vi "ExecuteCommand.vi"(0 "reference in":refnum<class "DqmhModuleDiagramGraph.lvclass">, 1 "CommandData":variant, 2 "selected":T1, 3 "selectedEdge":refnum<class "AbstractEdge.lvclass">, 4 "SelectedNodes":refnum<class "AbstractNode.lvclass">[](array[class]), 5 "error in (no error)":errorcluster) -> (14 "reference out":refnum<class "DqmhModuleDiagramGraph.lvclass">, 15 "Cancelled":bool, 19 "error out":errorcluster)   [LabVIEW 2020, in "DqmhModuleDiagramGraph.lvclass"]
uses:
  <resource>/Framework/Providers/Open_GDS/UML/DqmhModuleDiagramGraph_class/DqmhModuleDiagramGraph.lvclass
  <resource>/Framework/Providers/Open_GDS/UML/AbstractNode_class/AbstractNode.lvclass
  <resource>/Framework/Providers/Open_GDS/UML/AbstractEdge_class/AbstractEdge.lvclass
  <resource>/Framework/Providers/Open_GDS/UML/UMLEditor/UMLEditor tooltype.ctl
  <resource>/Framework/Providers/Open_GDS/UML/DQMHModuleNode_class/DQMHModuleNode.lvclass
  <resource>/Framework/Providers/Open_GDS/UML/DQMHModuleNode_class/ExternalSetTypes.ctl
  <resource>/Framework/Providers/Open_GDS/UML/DQMH_API_class/DQMH_API.lvclass
panel:
  out "StatusText":string
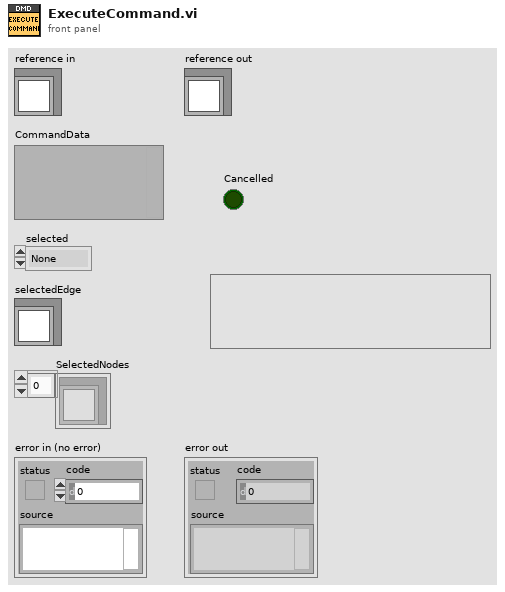
[diagram p1: front panel]
types:
  T1 = typedef "UMLEditor tooltype.ctl" = enum16{"None", "Node", "Edge"}
  T2 = enum32{"Invalid", "Standard", "Closed", "Hidden", "Minimized", "Maximized"}
  T3 = enum32{"Invalid", "Default", "Floating", "Floating/Auto-Hide", "Modal"}
  T4 = typedef "DQMHModuleNode.lvclass/ExternalSetTypes.ctl" = enum16{"Name", "Attributes", "Methods", "Position", "ShowEvents", "ShowInternalData", "ClassPath"}
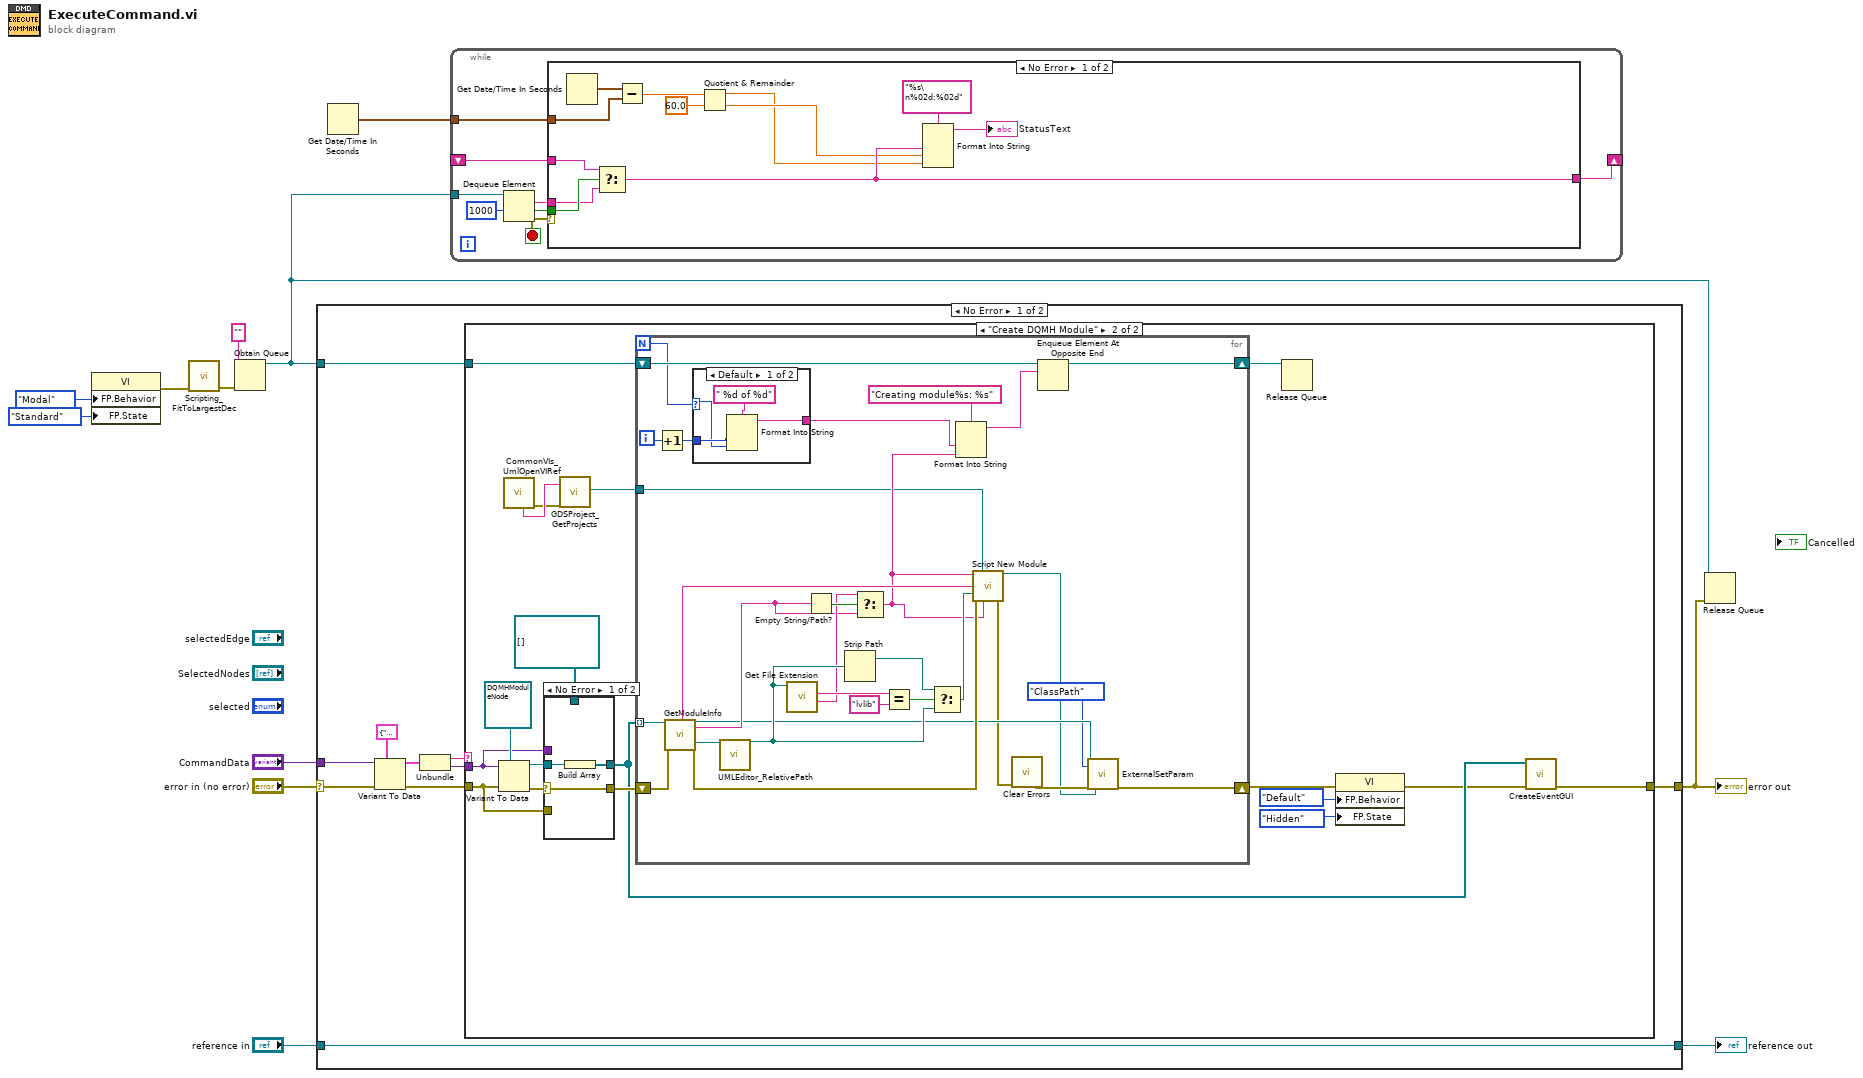
[diagram p0: block diagram]
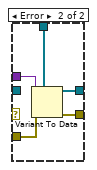
[diagram p4: hidden frame]
diagram:
  n1 = property class="VI"("FP.Behavior"=T3."Modal" ("Front Panel Window:Behavior"), "FP.State"=T2."Standard" ("Front Panel Window:State")) -> (error out=w2:errorcluster)  [unwired: 2 in, 1 out]
  n2 = call <resource>:"Scripting_FitToLargestDec.vi"("error in (no error)"=w2) -> ("error out"=w8:errorcluster)  [unwired: 5 in, 1 out]
  n3 = Obtain Queue(element data type="" ("y"), error in (no error)=w8) -> (queue out=w6:refnum<queue>)  [unwired: 3 in, 2 out]
  n4 = case shown="No Error" "error in (no error)" {
    selector: "error in (no error)" -> [w19 w85]
    tunnel: [w15 w85] -> w7
    tunnel: [w22 w84] -> w10
    tunnel: "reference in" -> [w22 w84]
    tunnel: "CommandData" -> [w20 _]
    tunnel: w6 -> [w13 _]
    frame No Error {
      n5 = Variant To Data(error in=w19, type=cluster{"Cmd":string, "Data":variant} {"Cmd"="", "Data"=variant} ("FlattenCommandSettings"), Variant=w20) -> (data=w18:cluster{"Cmd":string, "Data":variant}, error out=w16:errorcluster)
      n6 = Unbundle(w18) -> ("Cmd"=w17:string, "Data"=w14:variant)
      n7 = case shown="\"Create DQMH Module\"" w17 {
        tunnel: w16 -> [w23 w34]
        tunnel: [w23 w25] -> w15
        tunnel: w14 -> [_ w35]
        tunnel: w13 -> [_ w39]
        frame Default {
        }
        frame "Create DQMH Module" {
          n8 = Variant To Data(error in=w34, type=refnum<class "DQMHModuleNode.lvclass"> refnum ("DQMHModuleNode"), Variant=w35) -> (data=w40:refnum<class "DQMHModuleNode.lvclass">, error out=w38:errorcluster)
          n9 = call <resource>:"CommonVIs_UmlOpenVIRef.vi"() -> ("error out"=w32:errorcluster, "ProjectNameOut"=w33:string)  [unwired: 4 in, 6 out]
          n10 = case shown="No Error" w38 {
            selector: w38 -> [w42 _]
            tunnel: w40 -> [w44 _]
            tunnel: [w43 w45] -> w27
            tunnel: [w42 w46] -> w37
            tunnel: refnum<class "DQMHModuleNode.lvclass">[] [] -> [_ w49]
            tunnel: w35 -> [_ w48]
            tunnel: w34 -> [_ w47]
            frame No Error {
              n11 = Build Array(w44) -> (w43:refnum<class "DQMHModuleNode.lvclass">[])
            }
            frame Error {
              n12 = Variant To Data(error in=w47, type=w49, Variant=w48) -> (data=w45:refnum<class "DQMHModuleNode.lvclass">[], error out=w46:errorcluster)
            }
          }
          n13 = call <resource>:"GDSProject_GetProjects.vi"("GetProjectRefByName"=w33, "error in (no error)"=w32) -> ("Project Refnum"=w31:refnum<vi>)  [unwired: 1 in, 16 out]
          n14 = for {
            N -> [w62]
            tunnel: w27 -> [w63] mode=indexing
            shift-right: [w56] -> w28
            shift-left: w37 -> [w78]
            tunnel: w31 -> [w53]
            shift-right: [w50] -> w30
            shift-left: w39 -> [w64]
            i -> [w60]
            n15 = Increment(x=w60) -> (x+1=w61:i32)
            n16 = call-dynamic "GetModuleInfo.vi"("reference in"=w63, "error in (no error)"=w78) -> ("Template"=w75:string, "reference out"=w55:refnum<class "DQMHModuleNode.lvclass">, "ModuleName"=w67:string, "ModulePath"=w79:path, "error out"=w68:errorcluster)  [unwired: 6 in, 7 out]
            n17 = case shown="Default" w62 {
              selector: w62 -> [w81 _]
              tunnel: w61 -> [w82 _]
              tunnel: [w80 _] -> w59
              frame Default {
                n18 = Format Into String(format string=" %d of %d" ("element"), w82, w81) -> (resulting string=w80:string)  [unwired: 2 in, 1 out]
              }
              frame 1 {
              }
            }
            n19 = call <resource>:"UMLEditor_RelativePath.vi"("Path In"=w79) -> ("ConvertToAbsolutePath(If possible)"=w73:path)  [unwired: 1 in, 17 out]
            n20 = call <vilib>:"Get File Extension.vi"("file"=w73) -> ("filename without extension"=w69:string, "lowercase file extension"=w77:string)  [unwired: 6 in, 3 out]
            n21 = Empty String/Path?(string/path=w67) -> (empty?=w70:bool)
            n22 = Strip Path(path=w73) -> (stripped path=w72:path)  [unwired: 1 out]
            n23 = Select(t=w69, s=w70, f=w67) -> (s? t:f=w65:string)
            n24 = Equal?(x=w77, y="lvlib") -> (x = y?=w74:bool)
            n25 = Select(t=w72, s=w74, f=w73) -> (s? t:f=w71:path)
            n26 = Format Into String(format string="Creating module%s: %s" ("element"), w59, w65) -> (resulting string=w66:string)  [unwired: 2 in, 1 out]
            n27 = call <resource>:"Script New Module.vi"("Module Name"=w65, "Project"=w53, "ModuleType(String)"=w75, "Module Save Path"=w71, "error in (no error)"=w68, "Line 1 text"=w65) -> ("ModulePath(lvlib)"=w51:path, "error out"=w52:errorcluster)  [unwired: 8 in]
            n28 = call <vilib>:"Clear Errors.vi"("error in (no error)"=w52) -> ("error out"=w57:errorcluster)  [unwired: 5 in, 1 out]
            n29 = Enqueue Element At Opposite End(queue=w64, element=w66) -> (queue out=w50:refnum<queue>)  [unwired: 2 in, 2 out]
            n30 = call-dynamic "ExternalSetParam.vi"("reference in"=w55, "setParameter"=ExternalSetTypes."ClassPath", "error in (no error)"=w57, "ClassPath"=w51) -> ("error out"=w56:errorcluster)  [unwired: 14 in, 1 out]
          }
          n31 = Release Queue(queue=w30) -> ()  [unwired: 2 in, 3 out]
          n32 = property class="VI"(error in=w28, "FP.Behavior"=T3."Default" ("Front Panel Window:Behavior"), "FP.State"=T2."Hidden" ("Front Panel Window:State")) -> (error out=w26:errorcluster)  [unwired: 1 in, 1 out]
          n33 = call <resource>:"CreateEventGUI.vi"("error in (no error)"=w26, "DQMH_Modules"=w27) -> ("error out"=w25:errorcluster)  [unwired: 9 in]
        }
      }
    }
    frame Error {
    }
  }
  "error out" <- w7
  "reference out" <- w10
  n34 = Get Date/Time In Seconds() -> (seconds since 1Jan1904=w4:timestamp)
  n35 = while {
    tunnel: w6 -> [w93]
    tunnel: w4 -> [w90]
    shift-right: [w86] -> _
    shift-left: _ -> [w87]
    stop <- w92 stop-if-true
    n36 = Dequeue Element(queue=w93, timeout in ms (-1)=1000) -> (element=w89:string, timed out?=w88:bool, error out=w92:errorcluster)  [unwired: 1 in, 1 out]
    n37 = case shown="No Error" w92 {
      tunnel: w90 -> [w104 _]
      tunnel: w89 -> [w101 _]
      tunnel: w88 -> [w103 _]
      tunnel: w87 -> [w102 _]
      tunnel: [w99 _] -> w86
      frame No Error {
        n38 = Get Date/Time In Seconds() -> (seconds since 1Jan1904=w105:timestamp)
        n39 = Select(t=w102, s=w103, f=w101) -> (s? t:f=w99:string)
        n40 = Subtract(x=w105, y=w104) -> (x-y=w98:dbl)
        n41 = Quotient & Remainder(x=w98, y=60.0) -> (x-y*floor(x/y)=w95:dbl, floor(x/y)=w96:dbl)
        n42 = Format Into String(format string="%s\n%02d:%02d", w99, w96, w95) -> (resulting string=→"StatusText":string)  [unwired: 2 in, 1 out]
      }
      frame Error {
      }
    }
  }
  n43 = Release Queue(queue=w6, error in (no error)=w7) -> ()  [unwired: 1 in, 3 out]
